vi "Close.vi"(8 "error in (no error)":errorcluster, 11 "bt_Blackboard in":refnum<class "Blackboard.lvclass">) -> (0 "error out":errorcluster, 3 "bt_Blackboard out":refnum<class "Blackboard.lvclass">)   [LabVIEW 2021, in "Blackboard.lvclass"]
uses:
  Blackboard.lvclass
  Blackboard.lvclass/Blackboard.ctl
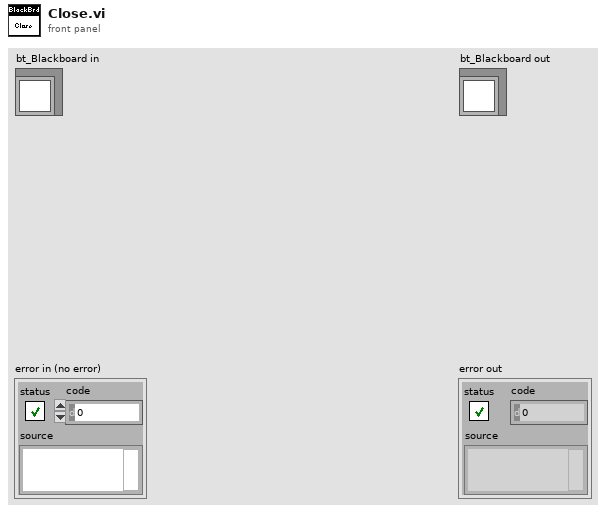
[diagram p1: front panel]
types:
  T1 = typedef "Blackboard.lvclass/Groups Type.ctl" = cluster{"Data":T2[], "Map":T5}
  T2 = typedef "Blackboard.lvclass/Data DVR Type.ctl" = cluster{"Tags":T3, "Data Refs":T4}
  T3 = typedef "Blackboard.lvclass/Tags Map Type.ctl" = map{string, refnum<class "Abs_Value.lvclass">}
  T4 = typedef "Local Bus.lvclass/Data Value References.ctl" = cluster{"Boolean":refnum<data-value>, "String":refnum<data-value>, "DBL":refnum<data-value>, "SGL":refnum<data-value>, "EXT":refnum<data-value>, "U8":refnum<data-value>, "U16":refnum<data-value>, "U32":refnum<data-value>, "U64":refnum<data-value>, "I8":refnum<data-value>, "I16":refnum<data-value>, "I32":refnum<data-value>, "I64":refnum<data-value>, "CDBL":refnum<data-value>, "CSGL":refnum<data-value>, "CEXT":refnum<data-value>, "Time":refnum<data-value>, "Variant":refnum<data-value>, "Waveform":refnum<data-value>, "Type":refnum<data-value>}
  T5 = typedef "Blackboard.lvclass/Group Map Type.ctl" = map{string, i32}
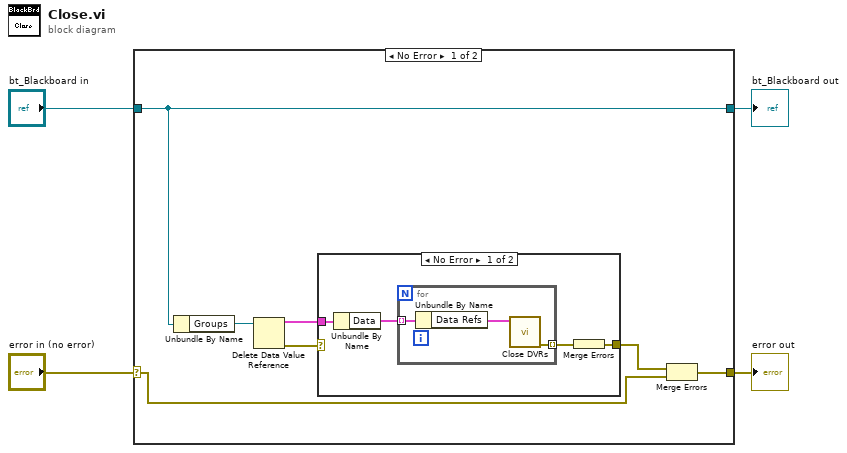
[diagram p0: block diagram]
diagram:
  n1 = case shown="No Error" "error in (no error)" {
    selector: "error in (no error)" -> [w6 w21]
    tunnel: [w5 w21] -> w3
    tunnel: [w10 w20] -> w1
    tunnel: "bt_Blackboard in" -> [w10 w20]
    frame No Error {
      n2 = Unbundle By Name(w10) -> ("Groups"=w11:refnum<data-value>)
      n3 = Delete Data Value Reference(data value reference=w11) -> (data value=w9:T1, error out=w8:errorcluster)  [unwired: 1 in]
      n4 = case shown="No Error" w8 {
        selector: w8 -> [_ w19]
        tunnel: [w13 w19] -> w7
        tunnel: w9 -> [w12 _]
        frame No Error {
          n5 = Unbundle By Name(w12) -> ("Data"=w15:T2[])
          n6 = for {
            tunnel: w15 -> [w17] mode=indexing
            tunnel: [w18] -> w14 mode=indexing
            n7 = Unbundle By Name(w17) -> ("Data Refs"=w16:T4)
            n8 = call "Close DVRs.vi"("Data Refs"=w16) -> ("error out"=w18:errorcluster)  [unwired: 10 in]
          }
          n9 = Merge Errors(w14) -> (w13:errorcluster)
        }
        frame Error {
        }
      }
      n10 = Merge Errors(w7, w6) -> (w5:errorcluster)
    }
    frame Error {
    }
  }
  "error out" <- w3
  "bt_Blackboard out" <- w1
